vi "Color Steps Control.vi"(7 "Calling VI Ref":refnum<vi>) -> ()   [LabVIEW 2016]
uses:
  <vilib>/Utility/miscctls.llb/LVPointTypeDef.ctl
  Color Steps Type Def/Color Steps Presets Type.ctl
  Color Steps Type Def/Color Steps Step Type.ctl
  Laser Control/Laser Power Control/Laser Power Control Type Defs/Laser Power Ctrl Base Type.ctl
  Color Steps Type Def/Color Steps Notifier Type.ctl
  Color Steps Type Def/Color Step Actions.ctl
  Hardware Configuration/Hardware Configuration Controls/Device Type.ctl
  Hardware Configuration/Hardware Configuration Controls/Device Function.ctl
  Device Library/Filter Wheels/FW Type Defs/FW Actions.ctl
  Laser Control/Laser Power Control/Laser Power Control Type Defs/Laser Power Ctrl Messenger Actions.ctl
panel:
  in  "Tab Control":enum32{"Step Control", "Setup"}(tab)
  in  "Presets":u16(ring) items=["None"]
  in  "Step":T1(radio)
  in  "Add Step":bool
  in  "Update Step":bool
  in  "Remove Step":bool
  in  "Clear All":bool
  in  "Preset_Name":string
  in  "Step_Name_01":string
  in  "Step_Name_02":string
  in  "Step_Name_03":string
  in  "Step_Name_04":string
  in  "Step_Name_05":string
  in  "Save Preset":bool
  in  "Setup":bool=TRUE
  in  "Quit":bool
  # "Preset Name:"
  # "Step 01 Name:"
  # "Step 04 Name:"
  # "Step 02 Name:"
  # "Step 05 Name:"
  # "Step 03 Name:"
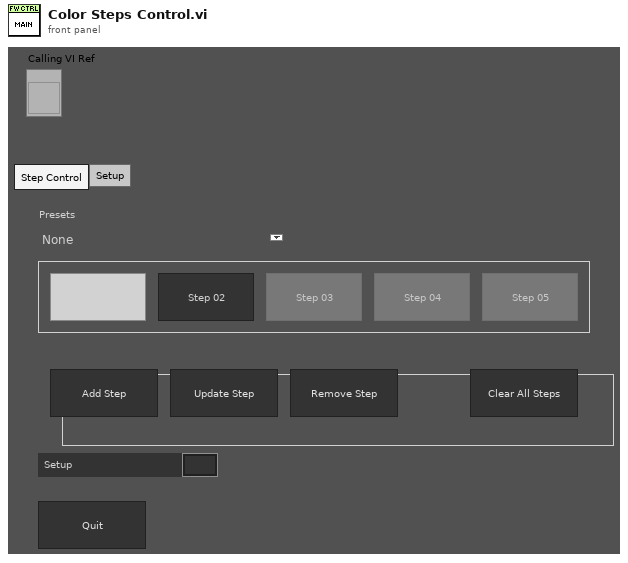
[diagram p1: front panel]
types:
  T1 = enum32{"Step 01", "Step 02", "Step 03", "Step 04", "Step 05"}
  T2 = typedef "Device Function.ctl" = enum16{"Primary", "Secondary", "Overview", "Wide Field Drift Correction", "642 nm Excitation", "560 nm Excitation", "940 nm Excitation", "546 nm Excitation", "488 nm Excitation", "405 nm Excitation", "Objective Drift Correction", "4Pi Objective Lock", "Objective XY", "Objective Z", "Sample XY", "Sample Coarse Z", "Sample Z", "4Pi Lower", "4Pi Upper", "Mojo", "Adj Cavity", "Line Scanning", "Alert"}
  T3 = typedef "Device Type.ctl" = enum16{"AOTF", "Camera", "Deformable Mirror", "Laser", "Shutter", "Stage", "Waveform", "FPGA", "Email", "Filter Wheel"}
  T4 = typedef "Color Steps Notifier Type.ctl" = cluster{"Actions":T5, "Set Step":i32, "Current Step":i32, "Last Step?":bool, "Received?":bool, "Preset Index":i32}
  T5 = typedef "Color Step Actions.ctl" = enum16{"Add Step", "Update Step", "Remove Step", "Clear All", "Get Status", "Next Step", "Go To Step", "Save Preset", "Change Preset", "Update Names", "Quit"}
  T6 = typedef "Color Steps Presets Type.ctl" = cluster{"Preset Name":string, "Steps":T7[]}
  T7 = typedef "Color Steps Step Type.ctl" = cluster{"Power Ctrl":T8[], "Filter Wheel Position":u8, "Step Name":string, "Wavelengths":u16[]}
  T8 = typedef "Laser Power Ctrl Base Type.ctl" = cluster{"Active":bool, "Power":dbl, "Ctrl Mode":u16}
  T9 = enum16{"Always On", "Always Off", "Off While Running"}
  T10 = typedef "LVPointTypeDef.ctl" = cluster{"Horizontal":i16, "Vertical":i16}
  T11 = enum8{"Enabled", "Disabled", "Disabled and Grayed Out"}
  T12 = typedef "LVRectTypeDef.ctl" = cluster{"Left":i16, "Top":i16, "Right":i16, "Bottom":i16}
  T13 = typedef "LVBoundsTypeDef.ctl" = cluster{"Width":u32, "Height":u32}
  T14 = typedef "Laser Power Ctrl Messenger Actions.ctl" = enum16{"All Active On", "All Off", "Adjust Power", "Line On/Off", "Get Status"}
  T15 = typedef "FW Actions.ctl" = enum16{"Set Position", "Get Position", "Get Num Positions", "Set Speed", "Quit"}
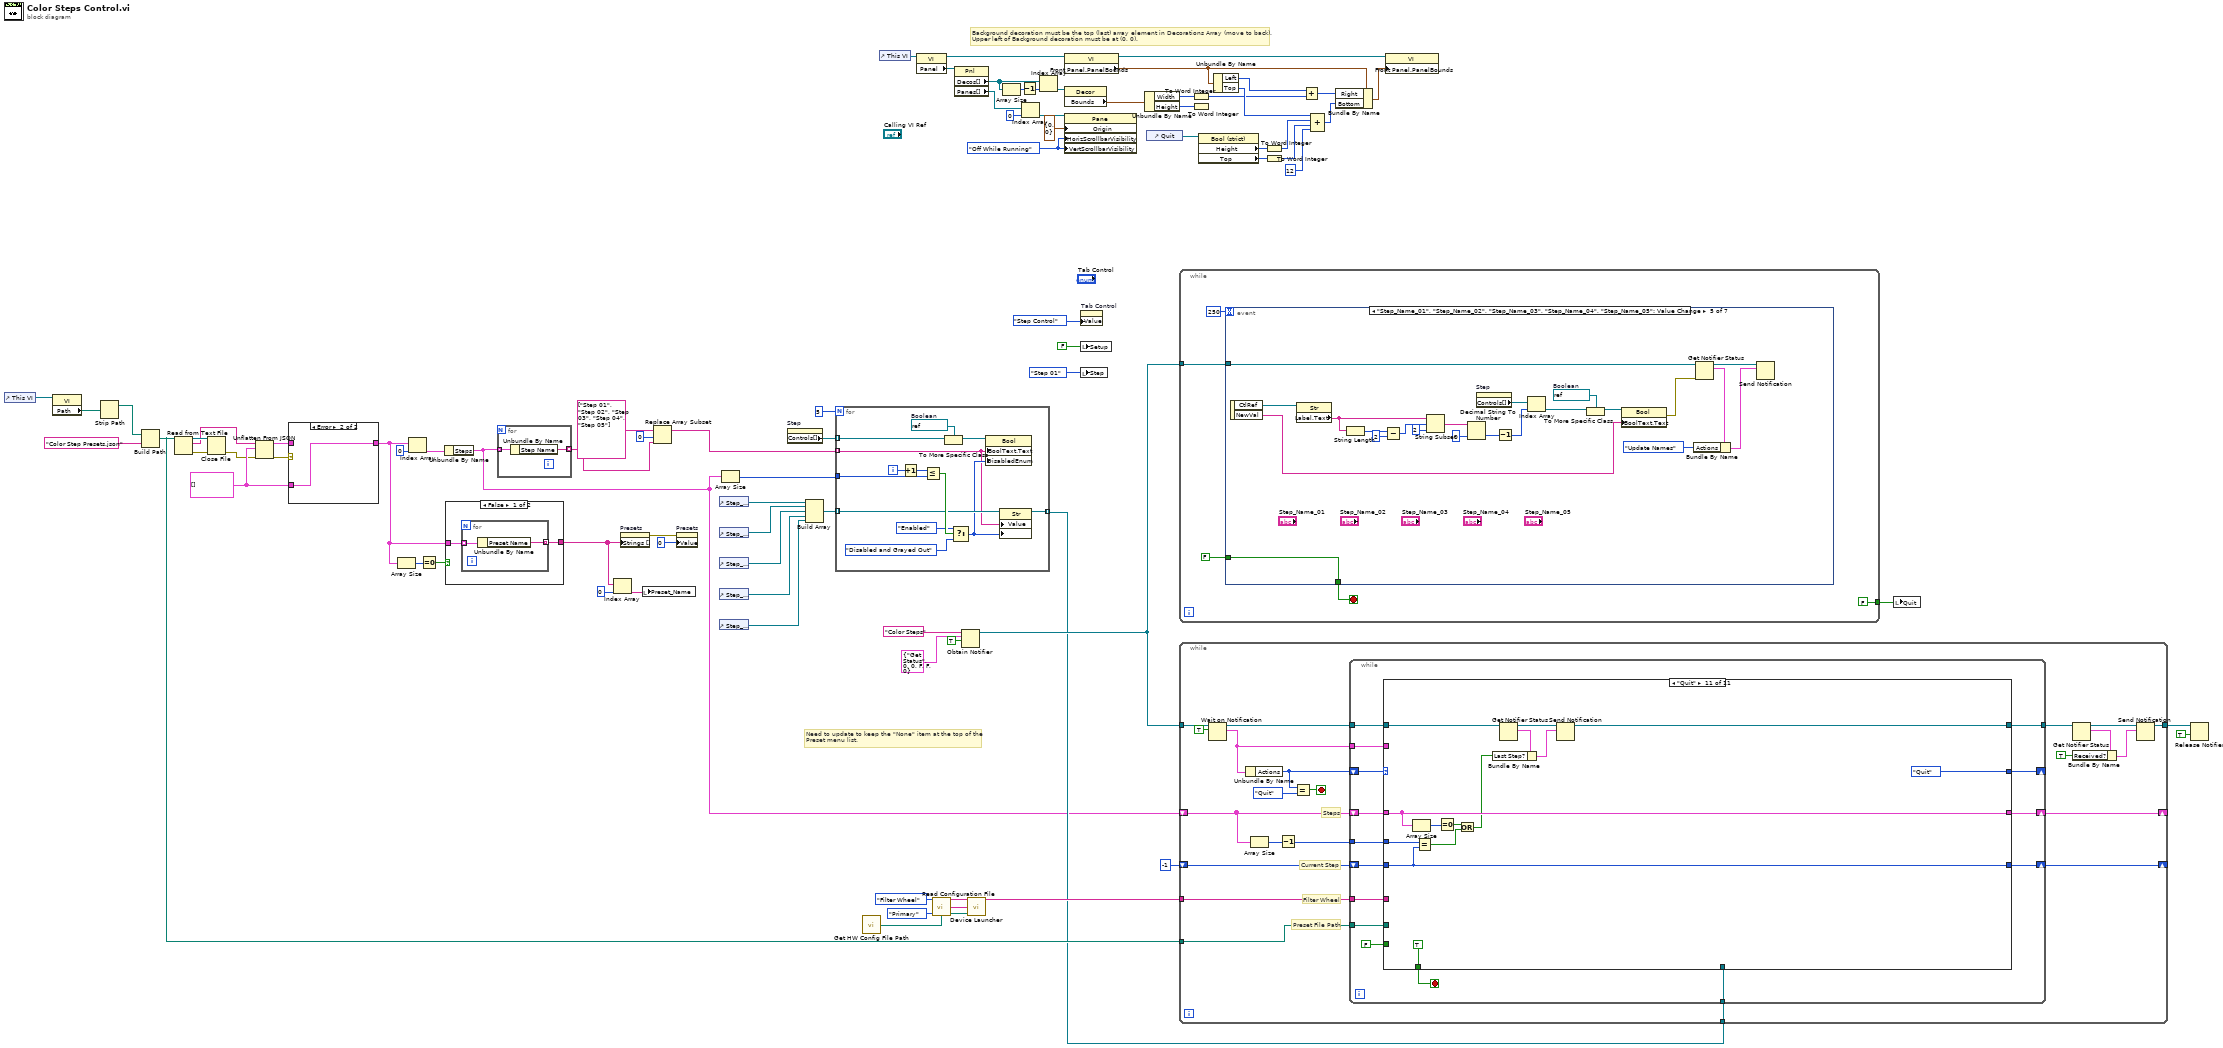
[diagram p0: block diagram]
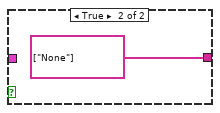
[diagram p2: hidden frame]
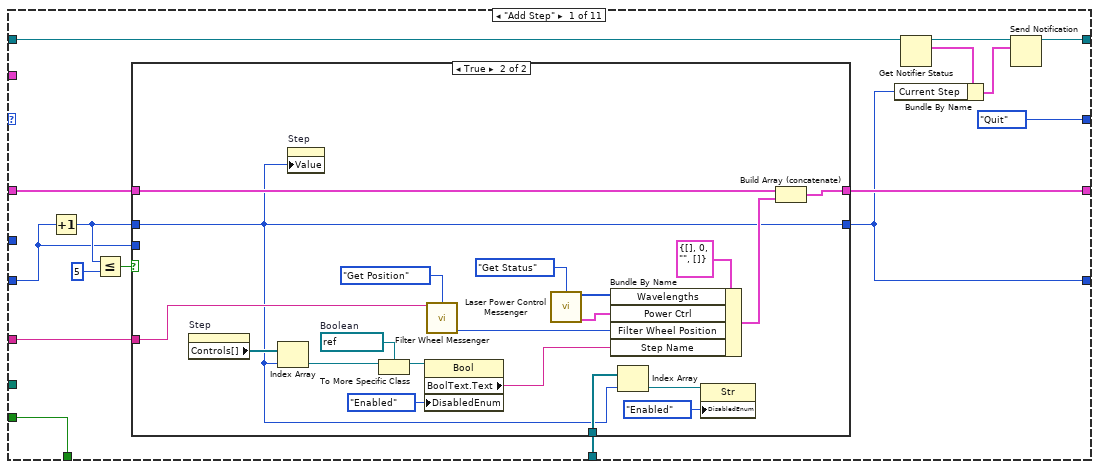
[diagram p3: hidden frame]
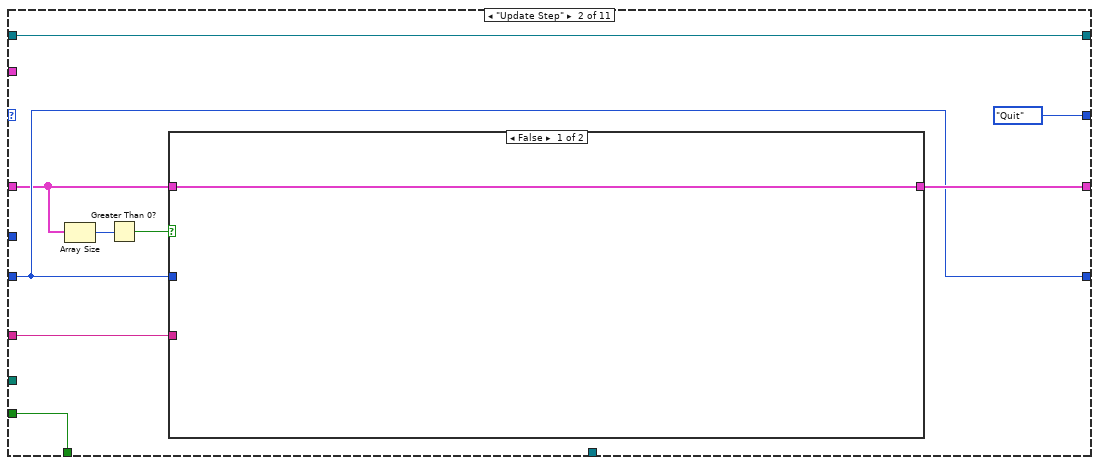
[diagram p5: hidden frame]
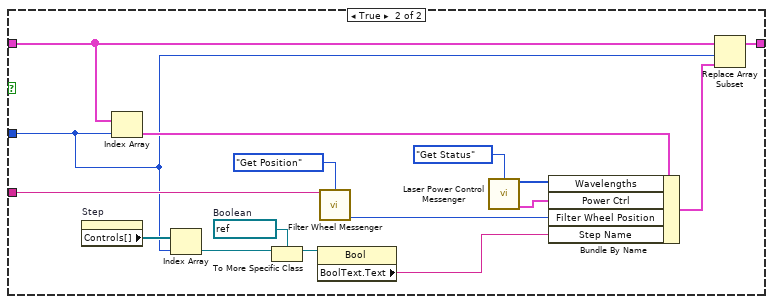
[diagram p6: hidden frame]
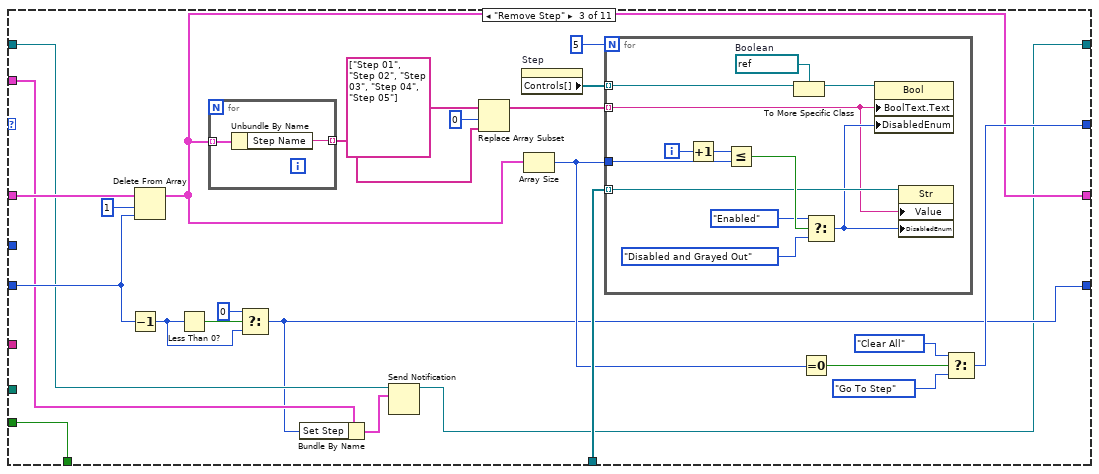
[diagram p7: hidden frame]
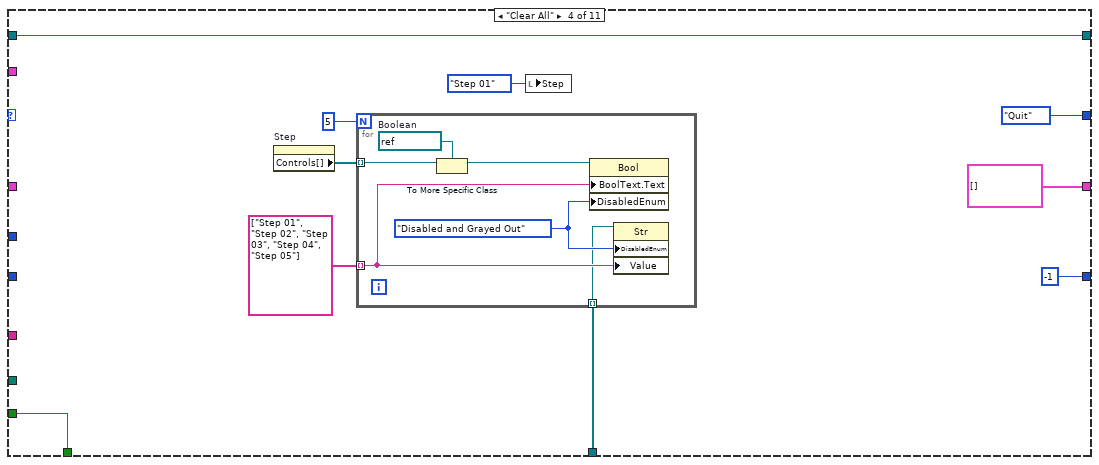
[diagram p8: hidden frame]
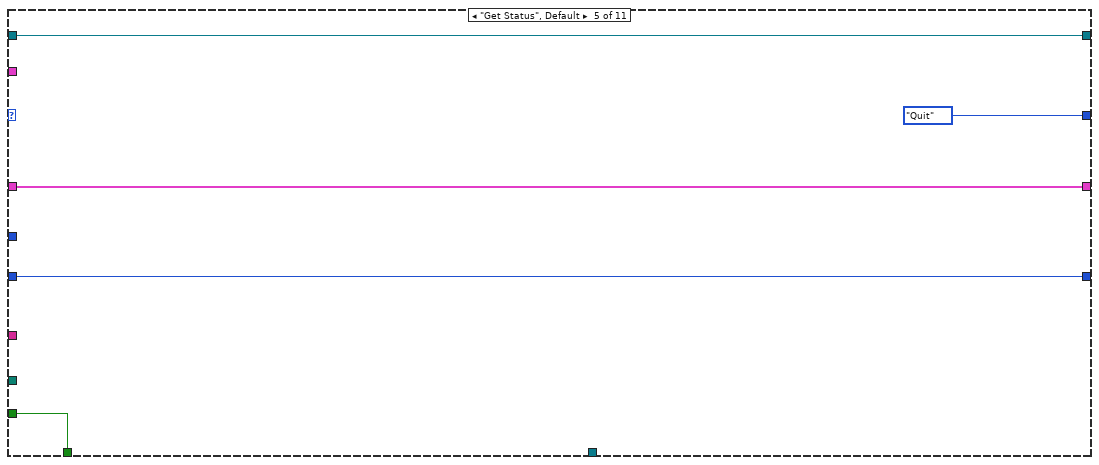
[diagram p9: hidden frame]
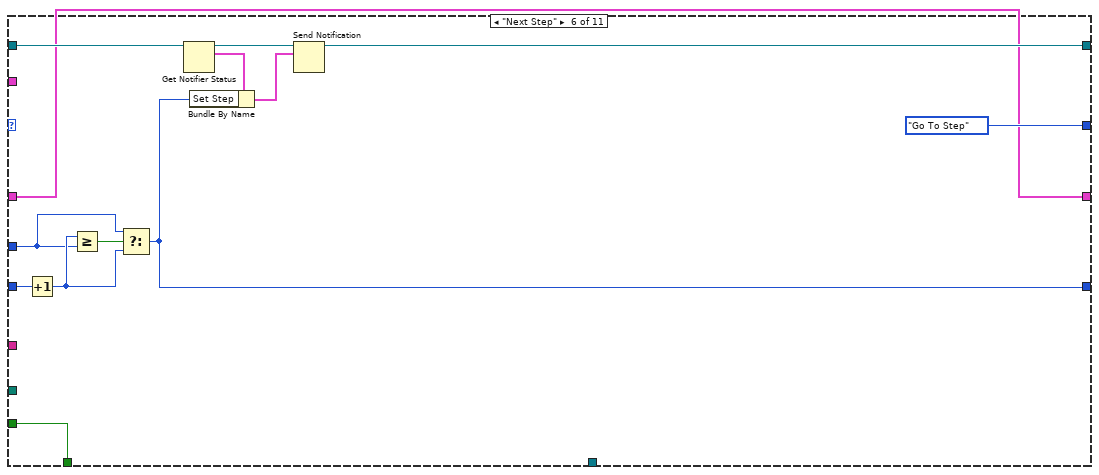
[diagram p10: hidden frame]
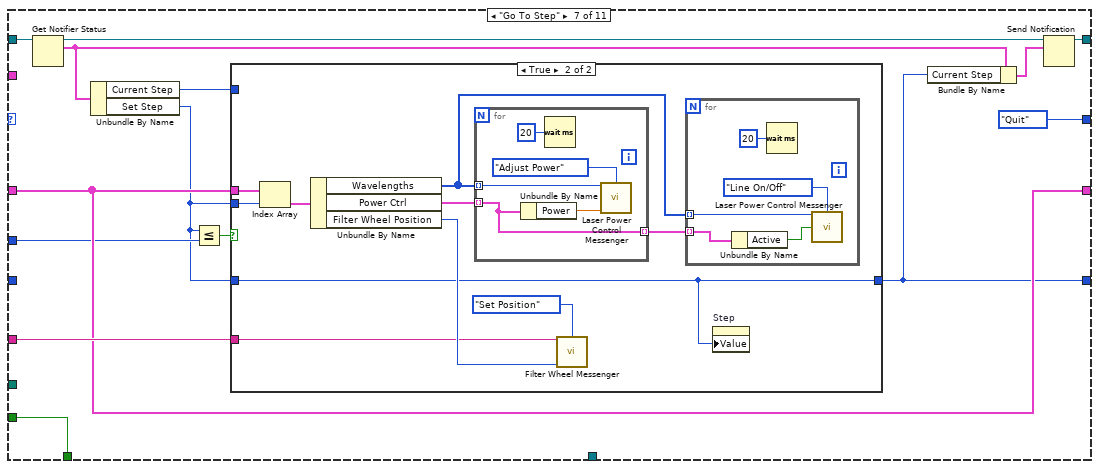
[diagram p11: hidden frame]
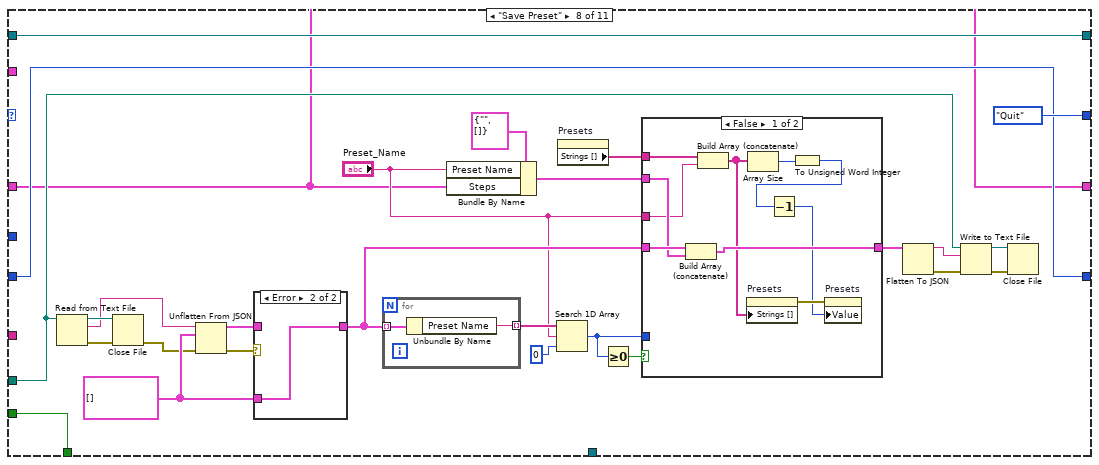
[diagram p13: hidden frame]
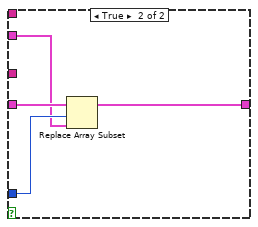
[diagram p14: hidden frame]
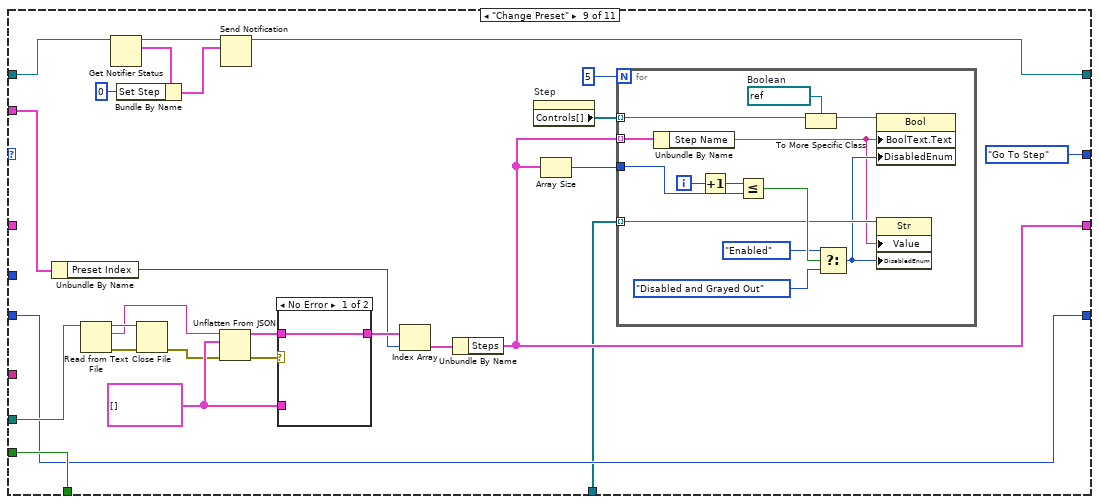
[diagram p16: hidden frame]
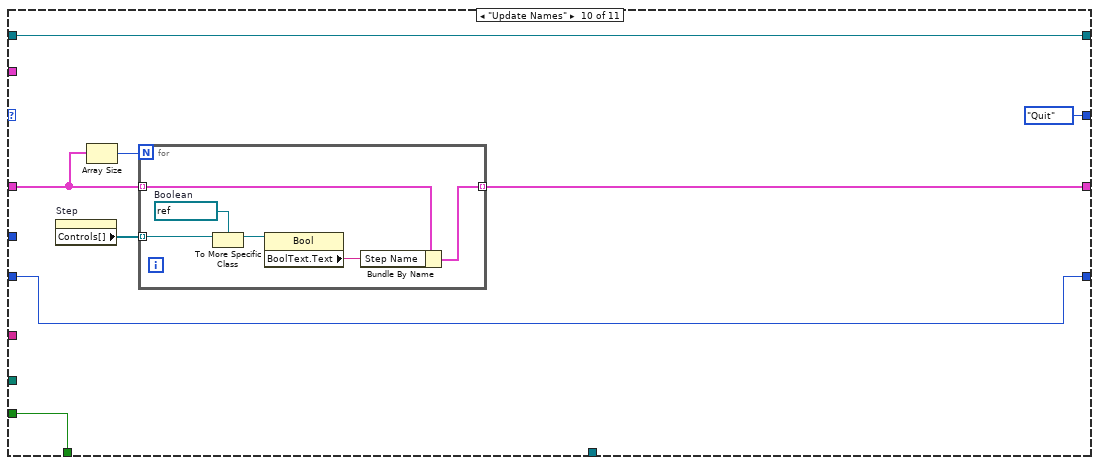
[diagram p18: hidden frame]
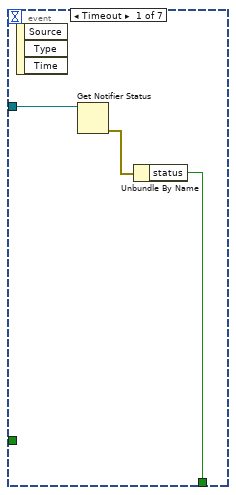
[diagram p19: hidden frame]
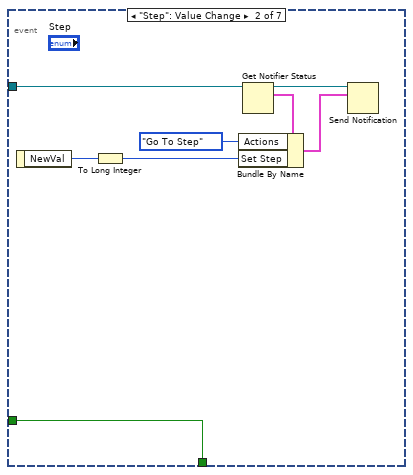
[diagram p20: hidden frame]
diagram:
  w40 = T6[] []
  w67 = T9."Off While Running" ("Vertical Scrollbar Visibility")
  # "Need to update to keep the \"None\" item at the top of the\nPreset menu list."
  # "Background decoration must be the top (last) array element in Decorations Array (move to back).\nUpper left of Background decoration must be at (0, 0)."
  n1 = control-ref of="This VI"() -> (w55:refnum<vi>)
  n2 = property class="VI"(reference=w55) -> ("Path"=w54:path)  [unwired: 1 in, 2 out]
  n3 = Strip Path(path=w54) -> (stripped path=w50:path)  [unwired: 1 out]
  n4 = Build Path(base path=w50, name or relative path="Color Step Presets.json") -> (appended path=w13:path)
  n5 = Read from Text File(file (use dialog)=w13) -> (refnum out=w39:refnum<file>, text=w36:string, error out=w38:errorcluster)  [unwired: 3 in, 1 out]
  n6 = Close File(refnum=w39, error in=w38) -> (error out=w37:errorcluster)  [unwired: 1 out]
  n7 = Unflatten From JSON(JSON string=w36, type and defaults=w40, error in (no error)=w37) -> (value=w51:T6[], error out=w52:errorcluster)  [unwired: 4 in]
  n8 = case shown="Error" w52 {
    tunnel: w51 -> [w85 _]
    tunnel: w40 -> [_ w86]
    tunnel: [w85 w86] -> w9
    frame No Error {
    }
    frame Error {
    }
  }
  n9 = Array Size(array=w9) -> (size(s)=w8:i32)
  n10 = Index Array(array=w9, index=0) -> (element=w23:T6)
  n11 = Equal To 0?(x=w8) -> (x = 0?=w7:bool)
  n12 = Unbundle By Name(w23) -> ("Steps"=w3:T7[])
  n13 = case shown="False" w7 {
    tunnel: w9 -> [w88 _]
    tunnel: [w87 string[] ["None"]] -> w11
    frame False {
      n14 = for {
        tunnel: w88 -> [w90] mode=indexing
        tunnel: [w89] -> w87 mode=indexing
        n15 = Unbundle By Name(w90) -> ("Preset Name"=w89:string)
      }
    }
    frame True {
    }
  }
  n16 = for {
    tunnel: w3 -> [w93] mode=indexing
    tunnel: [w92] -> w4 mode=indexing
    n17 = Unbundle By Name(w93) -> ("Step Name"=w92:string)
  }
  n18 = Index Array(array=w11, index=0) -> (element=w21:string)
  n19 = property on="Presets" class="Ring (strict)"("Strings []"=w11) -> (error out=w34:errorcluster)  [unwired: 2 in, 1 out]
  n20 = local write "Preset_Name"(w21) -> ()
  n21 = Replace Array Subset(array=string[] ["Step 01", "Step 02", "Step 03", "Step 04", "Step 05"], new element=w4, index=0) -> (w2:string[])
  n22 = property on="Presets" class="Ring (strict)"(error in=w34, "Value"=u16 0) -> ()  [unwired: 1 in, 2 out]
  n23 = control-ref of="Step_Name_01"() -> (w49:refnum<vi>)
  n24 = control-ref of="Step_Name_02"() -> (w45:refnum<vi>)
  n25 = control-ref of="Step_Name_03"() -> (w46:refnum<vi>)
  n26 = control-ref of="Step_Name_04"() -> (w47:refnum<vi>)
  n27 = control-ref of="Step_Name_05"() -> (w48:refnum<vi>)
  n28 = Array Size(array=w3) -> (size(s)=w32:i32)
  n29 = property on="Step" class="RadioBtnsControl (strict)"() -> ("Controls[]"=w43:refnum<vi>[])  [unwired: 2 in, 2 out]
  n30 = Build Array(w49, w45, w46, w47, w48) -> (w35:refnum<vi>[])
  n31 = for {
    N: 5 -> [_]
    tunnel: [w106] -> w12 mode=indexing
    tunnel: w43 -> [w105] mode=indexing
    tunnel: w35 -> [w97] mode=indexing
    tunnel: w32 -> [w96]
    tunnel: w2 -> [w94] mode=indexing
    i -> [w102]
    w104 = refnum<vi> refnum  # Boolean
    n32 = Increment(x=w102) -> (x+1=w101:i32)
    n33 = Less Or Equal?(x=w101, y=w96) -> (x <= y?=w100:bool)
    n34 = To More Specific Class(target class=w104, reference=w105) -> (specific class reference=w103:refnum<vi>)  [unwired: 1 in, 1 out]
    n35 = Select(t=T11."Enabled" ("Disabled"), s=w100, f=T11."Disabled and Grayed Out") -> (s? t:f=w95:T11)
    n36 = property class="Bool"(reference=w103, "BoolText.Text"=w94, "DisabledEnum"=w95) -> ()  [unwired: 1 in, 2 out]
    n37 = property class="Str"(reference=w97, "Value"=w94, "DisabledEnum"=w95) -> (reference out=w106:refnum<vi>)  [unwired: 1 in, 1 out]
  }
  n38 = call "Get HW Config File Path.vi"() -> ("File Path"=w15:path)  [unwired: 14 in, 1 out]
  n39 = control-ref of="This VI"() -> (w59:refnum<vi>)
  n40 = property class="VI"(reference=w59) -> (reference out=w68:refnum<vi>, "Panel"=w60:refnum<vi>)  [unwired: 1 in, 1 out]
  n41 = call "Read Configuration File.vi"("Device Type"=Device_Type."Filter Wheel", "Device Function"=Device_Function."Primary", "Config File Path"=w15) -> ("Unique Notifier Name"=w20:string, "Device Ports/IDs/Channels"=w18:string[], "Device Engine Path"=w19:path)  [unwired: 9 in, 1 out]
  n42 = property class="Pnl"(reference=w60) -> ("Decos[]"=w58:refnum<vi>[], "Panes[]"=w64:refnum<vi>[])  [unwired: 1 in, 2 out]
  n43 = Obtain Notifier(name (unnamed)="Color Steps", notification data type=T4 {"Actions"=enum."Get Status", "Set Step"=0, "Current Step"=0, "Last Step?"=FALSE, "Received?"=FALSE, "Preset Index"=0} ("Color Steps Note Type"), create if not found? (T)=TRUE) -> (notifier out=w27:refnum<notifier>)  [unwired: 1 in, 2 out]
  n44 = call "Device Launcher.vi"("Notifier Name"=w20, "Device Ports/IDs/Channels"=w18, "Device Engine Path"=w19) -> ("Notifier Name"=w14:string)  [unwired: 11 in, 1 out]
  n45 = Array Size(array=w58) -> (size(s)=w56:i32)
  n46 = Decrement(x=w56) -> (x-1=w57:i32)
  n47 = Index Array(array=w64, index=0) -> (element=w63:refnum<vi>)
  n48 = Index Array(array=w58, index=w57) -> (element=w66:refnum<vi>)
  n49 = property class="VI"(reference=w68) -> (reference out=w70:refnum<vi>, "Front Panel.PanelBounds"=w71:T12)  [unwired: 1 in, 1 out]
  n50 = property class="Decor"(reference=w66) -> ("Bounds"=w69:T13)  [unwired: 1 in, 2 out]
  n51 = property class="Pane"(reference=w63, "Origin"=T10 {"Horizontal"=0, "Vertical"=0}, "HorizScrollbarVisibility"=w67, "VertScrollbarVisibility"=w67) -> ()  [unwired: 1 in, 2 out]
  n52 = property on="Tab Control" class="TabCtl (strict)"("Value"=enum32{"Step Control", "Setup"}."Step Control" ("Tab Control")) -> ()  [unwired: 2 in, 2 out]
  n53 = local write "Setup"(FALSE ("Filter Wheel Setup")) -> ()
  n54 = local write "Step"(T1."Step 01" ("Step")) -> ()
  n55 = Unbundle By Name(w69) -> ("Width"=w74:u32, "Height"=w77:u32)
  n56 = control-ref of="Quit"() -> (w61:refnum<vi>)
  n57 = while {
    tunnel: w27 -> [w108]
    tunnel: [FALSE] -> w1
    stop <- w110 stop-if-true
    n58 = event shown="[4] \"Step_Name_01\", \"Step_Name_02\", \"Step_Name_03\", \"Step_Name_04\", \"Step_Name_05\": Value Change" {
      selector: _ -> [_ _ _ _ _ _ _]
      dyn-events: _ -> [_ _ _ _ _ _ _]
      timeout: 250 -> [_ _ _ _ _ _ _]
      tunnel: FALSE -> [_ w122 w130 w141 w163 w171 _]
      tunnel: [w112 w122 w130 w141 w163 w171 w177] -> w110
      tunnel: w108 -> [w114 w121 w124 _ w143 w166 w172]
      event Timeout {
        n59 = event-data() -> ()  [unwired: 1 in, 3 out]
        n60 = Get Notifier Status(notifier=w114) -> (error out=w113:errorcluster)  [unwired: 1 in, 4 out]
        n61 = Unbundle By Name(w113) -> ("status"=w112:bool)
      }
      event "Step": Value Change {
        n62 = event-data() -> ("NewVal"=w116:T1)  [unwired: 1 in]
        n63 = To Long Integer(number=w116) -> (32bit integer=w115:i32)
        n64 = Get Notifier Status(notifier=w121) -> (notifier out=w120:refnum<notifier>, current notification=w119:T4)  [unwired: 1 in, 3 out]
        n65 = Bundle By Name(cluster=w119, "Actions"=Color_Step_Actions."Go To Step", "Set Step"=w115) -> (w117:T4)
        n66 = Send Notification(notification=w117, notifier=w120) -> ()  [unwired: 1 in, 2 out]
      }
      event "Add Step", "Update Step", "Remove Step", "Clear All", "Save Preset": Value Change {
        n67 = event-data() -> ("CtlRef"=w129:refnum<vi>)  [unwired: 1 in]
        n68 = property class="Bool"(reference=w129) -> ("Label.Text"=w128:string)  [unwired: 1 in, 2 out]
        n69 = case shown="\"Add Step\"" w128 {
          tunnel: [Color_Step_Actions."Get Status" ("Actions") Color_Step_Actions."Add Step" ("Actions") Color_Step_Actions."Update Step" ("Actions") Color_Step_Actions."Remove Step" ("Actions") Color_Step_Actions."Clear All" ("Actions") Color_Step_Actions."Save Preset" ("Actions")] -> w123
          frame Default {
          }
          frame "Add Step" {
          }
          frame "Update Step" {
          }
          frame "Remove Step" {
          }
          frame "Clear All" {
          }
          frame "Save Preset" {
          }
        }
        n70 = Get Notifier Status(notifier=w124) -> (notifier out=w127:refnum<notifier>, current notification=w126:T4)  [unwired: 1 in, 3 out]
        n71 = Bundle By Name(cluster=w126, "Actions"=w123) -> (w125:T4)
        n72 = Send Notification(notification=w125, notifier=w127) -> ()  [unwired: 1 in, 2 out]
      }
      event "Setup": Value Change {
        n73 = event-data() -> ("NewVal"=w140:bool)  [unwired: 1 in]
        n74 = Select(t=enum32{"Step Control", "Setup"}."Setup" ("Tab Control"), s=w140, f=enum32{"Step Control", "Setup"}."Step Control" ("Tab Control")) -> (s? t:f=w137:enum32{"Step Control", "Setup"})
        n75 = property on="Tab Control" class="TabCtl (strict)"("Value"=w137) -> ()  [unwired: 2 in, 2 out]
      }
      event "Step_Name_01", "Step_Name_02", "Step_Name_03", "Step_Name_04", "Step_Name_05": Value Change {
        w162 = refnum<vi> refnum  # Boolean
        n76 = event-data() -> ("CtlRef"=w149:refnum<vi>, "NewVal"=w148:string)  [unwired: 1 in]
        n77 = property class="Str"(reference=w149) -> ("Label.Text"=w160:string)  [unwired: 1 in, 2 out]
        n78 = String Length(string=w160) -> (length=w159:i32)
        n79 = Subtract(x=w159, y=2) -> (x-y=w157:i32)
        n80 = String Subset(string=w160, offset (0)=w157, length (rest)=2 ("length (rest)")) -> (substring=w156:string)
        n81 = Decimal String To Number(string=w156, default (0L)=0 ("default (0 I32)")) -> (number=w153:i32)  [unwired: 1 in, 1 out]
        n82 = property on="Step" class="RadioBtnsControl (strict)"() -> ("Controls[]"=w154:refnum<vi>[])  [unwired: 2 in, 2 out]
        n83 = Decrement(x=w153) -> (x-1=w150:i32)
        n84 = Index Array(array=w154, index=w150) -> (element=w152:refnum<vi>)
        n85 = To More Specific Class(target class=w162, reference=w152) -> (specific class reference=w151:refnum<vi>)  [unwired: 1 in, 1 out]
        n86 = property class="Bool"(reference=w151, "BoolText.Text"=w148) -> (error out=w142:errorcluster)  [unwired: 1 in, 1 out]
        n87 = Get Notifier Status(notifier=w143, error in (no error)=w142) -> (notifier out=w147:refnum<notifier>, current notification=w146:T4)  [unwired: 3 out]
        n88 = Bundle By Name(cluster=w146, "Actions"=Color_Step_Actions."Update Names") -> (w144:T4)
        n89 = Send Notification(notification=w144, notifier=w147) -> ()  [unwired: 1 in, 2 out]
      }
      event "Presets": Value Change {
        n90 = event-data() -> ("NewVal"=w165:u16)  [unwired: 1 in]
        n91 = To Long Integer(number=w165) -> (32bit integer=w164:i32)
        n92 = Get Notifier Status(notifier=w166) -> (notifier out=w170:refnum<notifier>, current notification=w169:T4)  [unwired: 1 in, 3 out]
        n93 = Bundle By Name(cluster=w169, "Actions"=Color_Step_Actions."Change Preset", "Preset Index"=w164) -> (w167:T4)
        n94 = Send Notification(notification=w167, notifier=w170) -> ()  [unwired: 1 in, 2 out]
      }
      event "Quit": Value Change {
        n95 = event-data() -> ("NewVal"=w177:bool)  [unwired: 1 in]
        n96 = Get Notifier Status(notifier=w172) -> (notifier out=w176:refnum<notifier>, current notification=w175:T4)  [unwired: 1 in, 3 out]
        n97 = Bundle By Name(cluster=w175, "Actions"=Color_Step_Actions."Quit") -> (w173:T4)
        n98 = Send Notification(notification=w173, notifier=w176) -> ()  [unwired: 1 in, 2 out]
      }
    }
  }
  n99 = while {
    tunnel: w27 -> [w199]
    shift-right: [w185] -> _
    shift-left: w3 -> [w192]
    tunnel: [w178] -> w26
    shift-right: [w188] -> _
    shift-left: -1 -> [w193]
    tunnel: w14 -> [w189]
    tunnel: w13 -> [w187]
    tunnel: w12 -> [w184]
    stop <- w196 stop-if-true
    # "Preset File Path"
    # "Filter Wheel"
    # "Steps"
    # "Current Step"
    n100 = Wait on Notification(notifier=w199, ignore previous (F)=TRUE) -> (notifier out=w195:refnum<notifier>, notification=w186:T4)  [unwired: 2 in, 2 out]
    n101 = Unbundle By Name(w186) -> ("Actions"=w194:T5)
    n102 = Array Size(array=w192) -> (size(s)=w191:i32)
    n103 = Decrement(x=w191) -> (x-1=w190:i32)
    n104 = Equal?(x=w194, y=Color_Step_Actions."Quit") -> (x = y?=w196:bool)
    n105 = while {
      tunnel: w195 -> [w214]
      shift-right: [w206] -> _
      shift-left: w194 -> [w213]
      shift-right: [w201] -> w188
      shift-left: w193 -> [w208]
      shift-right: [w203] -> w185
      shift-left: w192 -> [w209]
      tunnel: w190 -> [w210]
      tunnel: w189 -> [w207]
      tunnel: w187 -> [w205]
      tunnel: w186 -> [w204]
      tunnel: w184 -> [w202]
      tunnel: [w200] -> w179
      stop <- w211 stop-if-true
      n106 = case shown="\"Quit\"" w213 {
        tunnel: w214 -> [w222 w256 w282 w326 w337 w346 w354 w390 w434 w479 w495]
        tunnel: FALSE -> [w230 w261 w303 w327 w338 w351 w365 w413 w457 w480 _]
        tunnel: [w230 w261 w303 w327 w338 w351 w365 w413 w457 w480 TRUE] -> w211
        tunnel: [w221 w256 w279 w326 w337 w345 w362 w390 w432 w479 w494] -> w200
        tunnel: w210 -> [_ _ _ _ _ w341 w359 _ _ _ w493]
        tunnel: w209 -> [w229 w255 w302 _ w334 w340 w360 w387 _ w476 w491]
        tunnel: w208 -> [w216 w258 w300 _ w336 w350 _ w392 w444 w473 w492]
        tunnel: w207 -> [w226 w260 _ _ _ _ w364 _ _ _ _]
        tunnel: [w220 w258 w280 -1 ("Set Step") w336 w339 w355 w392 w444 w473 w492] -> w201
        tunnel: [Color_Step_Actions."Quit" ("y") Color_Step_Actions."Quit" ("y") w287 Color_Step_Actions."Quit" ("y") Color_Step_Actions."Quit" ("y") Color_Step_Actions."Go To Step" ("y") Color_Step_Actions."Quit" ("y") Color_Step_Actions."Quit" ("y") Color_Step_Actions."Go To Step" ("y") Color_Step_Actions."Quit" ("y") Color_Step_Actions."Quit" ("y")] -> w206
        tunnel: w205 -> [_ _ _ _ _ _ _ w395 w449 _ _]
        tunnel: w204 -> [_ _ w283 _ _ _ _ _ w448 _ _]
        tunnel: [w227 w259 w286 T7[] [] ("Steps") w334 w340 w360 w387 w440 w477 w491] -> w203
        tunnel: w202 -> [w215 _ w295 w320 _ _ _ _ w438 _ _]
        frame "Add Step" {
          n107 = Increment(x=w216) -> (x+1=w218:i32)
          n108 = Less Or Equal?(x=w218, y=5) -> (x <= y?=w219:bool)
          n109 = case shown="True" w219 {
            tunnel: w229 -> [w232 w252]
            tunnel: [w232 w251] -> w227
            tunnel: w226 -> [_ w240]
            tunnel: w218 -> [_ w233]
            tunnel: [w231 w233] -> w220
            tunnel: w216 -> [w231 _]
            tunnel: w215 -> [_ w236]
            frame False {
            }
            frame True {
              w249 = refnum<vi> refnum  # Boolean
              n110 = property on="Step" class="RadioBtnsControl (strict)"() -> ("Controls[]"=w250:refnum<vi>[])  [unwired: 2 in, 2 out]
              n111 = Index Array(array=w250, index=w233) -> (element=w248:refnum<vi>)
              n112 = property on="Step" class="RadioBtnsControl (strict)"("Value"=w233) -> ()  [unwired: 2 in, 2 out]
              n113 = To More Specific Class(target class=w249, reference=w248) -> (specific class reference=w247:refnum<vi>)  [unwired: 1 in, 1 out]
              n114 = property class="Bool"(reference=w247, "DisabledEnum"=T11."Enabled" ("Disabled")) -> ("BoolText.Text"=w246:string)  [unwired: 1 in, 2 out]
              n115 = call "Filter Wheel Messenger.vi"("FW Notifier"=w240, "Actions"=FW_Actions."Get Position") -> ("Current Position"=w244:u8)  [unwired: 11 in, 2 out]
              n116 = call "Laser Power Control Messenger.vi"("Power Ctrl Actions"=Laser_Power_Ctrl_Messenger_Actions."Get Status") -> ("Wavelengths"=w242:u16[], "Power Status"=w241:T8[])  [unwired: 13 in]
              n117 = Bundle By Name(cluster=T7 {"Power Ctrl"=[], "Filter Wheel Position"=0, "Step Name"="", "Wavelengths"=[]} ("Step"), "Wavelengths"=w242, "Power Ctrl"=w241, "Filter Wheel Position"=w244, "Step Name"=w246) -> (w238:T7)
              n118 = Index Array(array=w236, index=w233) -> (element=w235:refnum<vi>)
              n119 = property class="Str"(reference=w235, "DisabledEnum"=T11."Enabled" ("Disabled")) -> ()  [unwired: 1 in, 2 out]
              n120 = Build Array (concatenate)(w252, w238) -> (w251:T7[])
            }
          }
          n121 = Get Notifier Status(notifier=w222) -> (notifier out=w223:refnum<notifier>, current notification=w224:T4)  [unwired: 1 in, 3 out]
          n122 = Bundle By Name(cluster=w224, "Current Step"=w220) -> (w225:T4)
          n123 = Send Notification(notification=w225, notifier=w223) -> (notifier out=w221:refnum<notifier>)  [unwired: 1 in, 1 out]
        }
        frame "Update Step" {
          n124 = Array Size(array=w255) -> (size(s)=w254:i32)
          n125 = Greater Than 0?(x=w254) -> (x > 0?=w253:bool)
          n126 = case shown="False" w253 {
            tunnel: w260 -> [_ w270]
            tunnel: [w262 w265] -> w259
            tunnel: w258 -> [_ w264]
            tunnel: w255 -> [w262 w263]
            frame False {
            }
            frame True {
              w275 = refnum<vi> refnum  # Boolean
              n127 = property on="Step" class="RadioBtnsControl (strict)"() -> ("Controls[]"=w276:refnum<vi>[])  [unwired: 2 in, 2 out]
              n128 = Index Array(array=w263, index=w264) -> (element=w278:T7)
              n129 = Index Array(array=w276, index=w264) -> (element=w274:refnum<vi>)
              n130 = To More Specific Class(target class=w275, reference=w274) -> (specific class reference=w273:refnum<vi>)  [unwired: 1 in, 1 out]
              n131 = property class="Bool"(reference=w273) -> ("BoolText.Text"=w272:string)  [unwired: 1 in, 2 out]
              n132 = call "Filter Wheel Messenger.vi"("FW Notifier"=w270, "Actions"=FW_Actions."Get Position") -> ("Current Position"=w269:u8)  [unwired: 11 in, 2 out]
              n133 = call "Laser Power Control Messenger.vi"("Power Ctrl Actions"=Laser_Power_Ctrl_Messenger_Actions."Get Status") -> ("Wavelengths"=w267:u16[], "Power Status"=w266:T8[])  [unwired: 13 in]
              n134 = Bundle By Name(cluster=w278, "Wavelengths"=w267, "Power Ctrl"=w266, "Filter Wheel Position"=w269, "Step Name"=w272) -> (w277:T7)
              n135 = Replace Array Subset(array=w263, new element=w277, index=w264) -> (w265:T7[])
            }
          }
        }
        frame "Remove Step" {
          n136 = Decrement(x=w300) -> (x-1=w299:i32)
          n137 = Delete From Array(array=w302, length=1, index=w300) -> (array with subset deleted=w286:T7[])  [unwired: 1 out]
          n138 = Less Than 0?(x=w299) -> (x < 0?=w288:bool)
          n139 = for {
            tunnel: w286 -> [w305] mode=indexing
            tunnel: [w304] -> w292 mode=indexing
            n140 = Unbundle By Name(w305) -> ("Step Name"=w304:string)
          }
          n141 = Select(t=0, s=w288, f=w299) -> (s? t:f=w280:i32)
          n142 = Bundle By Name(cluster=w283, "Set Step"=w280) -> (w281:T4)
          n143 = Send Notification(notification=w281, notifier=w282) -> (notifier out=w279:refnum<notifier>)  [unwired: 1 in, 1 out]
          n144 = Replace Array Subset(array=string[] ["Step 01", "Step 02", "Step 03", "Step 04", "Step 05"], new element=w292, index=0) -> (w291:string[])
          n145 = property on="Step" class="RadioBtnsControl (strict)"() -> ("Controls[]"=w296:refnum<vi>[])  [unwired: 2 in, 2 out]
          n146 = Array Size(array=w286) -> (size(s)=w285:i32)
          n147 = for {
            N: 5 -> [_]
            tunnel: w296 -> [w317] mode=indexing
            tunnel: w295 -> [w309] mode=indexing
            tunnel: w285 -> [w308]
            tunnel: w291 -> [w306] mode=indexing
            i -> [w314]
            w316 = refnum<vi> refnum  # Boolean
            n148 = Increment(x=w314) -> (x+1=w313:i32)
            n149 = Less Or Equal?(x=w313, y=w308) -> (x <= y?=w312:bool)
            n150 = To More Specific Class(target class=w316, reference=w317) -> (specific class reference=w315:refnum<vi>)  [unwired: 1 in, 1 out]
            n151 = Select(t=T11."Enabled" ("Disabled"), s=w312, f=T11."Disabled and Grayed Out") -> (s? t:f=w307:T11)
            n152 = property class="Bool"(reference=w315, "BoolText.Text"=w306, "DisabledEnum"=w307) -> ()  [unwired: 1 in, 2 out]
            n153 = property class="Str"(reference=w309, "Value"=w306, "DisabledEnum"=w307) -> ()  [unwired: 1 in, 2 out]
          }
          n154 = Equal To 0?(x=w285) -> (x = 0?=w284:bool)
          n155 = Select(t=Color_Step_Actions."Clear All" ("y"), s=w284, f=Color_Step_Actions."Go To Step" ("y")) -> (s? t:f=w287:T5)
        }
        frame "Clear All" {
          n156 = property on="Step" class="RadioBtnsControl (strict)"() -> ("Controls[]"=w322:refnum<vi>[])  [unwired: 2 in, 2 out]
          n157 = for {
            N: 5 -> [_]
            tunnel: w322 -> [w333] mode=indexing
            tunnel: string[] ["Step 01", "Step 02", "Step 03", "Step 04", "Step 05"] -> [w329] mode=indexing
            tunnel: w320 -> [w328] mode=indexing
            w330 = T11."Disabled and Grayed Out" ("f")
            w332 = refnum<vi> refnum  # Boolean
            n158 = To More Specific Class(target class=w332, reference=w333) -> (specific class reference=w331:refnum<vi>)  [unwired: 1 in, 1 out]
            n159 = property class="Bool"(reference=w331, "BoolText.Text"=w329, "DisabledEnum"=w330) -> ()  [unwired: 1 in, 2 out]
            n160 = property class="Str"(reference=w328, "DisabledEnum"=w330, "Value"=w329) -> ()  [unwired: 1 in, 2 out]
          }
          n161 = local write "Step"(T1."Step 01" ("Step")) -> ()
        }
        frame "Get Status", Default {
        }
        frame "Next Step" {
          n162 = Increment(x=w350) -> (x+1=w343:i32)
          n163 = Greater Or Equal?(x=w343, y=w341) -> (x >= y?=w342:bool)
          n164 = Select(t=w341, s=w342, f=w343) -> (s? t:f=w339:i32)
          n165 = Get Notifier Status(notifier=w346) -> (notifier out=w347:refnum<notifier>, current notification=w348:T4)  [unwired: 1 in, 3 out]
          n166 = Bundle By Name(cluster=w348, "Set Step"=w339) -> (w349:T4)
          n167 = Send Notification(notification=w349, notifier=w347) -> (notifier out=w345:refnum<notifier>)  [unwired: 1 in, 1 out]
        }
        frame "Go To Step" {
          n168 = Get Notifier Status(notifier=w354) -> (notifier out=w353:refnum<notifier>, current notification=w352:T4)  [unwired: 1 in, 3 out]
          n169 = Unbundle By Name(w352) -> ("Current Step"=w356:i32, "Set Step"=w357:i32)
          n170 = Less Or Equal?(x=w357, y=w359) -> (x <= y?=w358:bool)
          n171 = case shown="True" w358 {
            tunnel: w364 -> [_ w370]
            tunnel: w357 -> [_ w369]
            tunnel: w360 -> [_ w368]
            tunnel: w357 -> [_ w367]
            tunnel: [w366 w367] -> w355
            tunnel: w356 -> [w366 _]
            frame False {
            }
            frame True {
              n172 = Index Array(array=w368, index=w369) -> (element=w371:T7)
              n173 = Unbundle By Name(w371) -> ("Wavelengths"=w376:u16[], "Power Ctrl"=w374:T8[], "Filter Wheel Position"=w373:u8)
              n174 = for {
                tunnel: w374 -> [w383] mode=indexing
                tunnel: w376 -> [w384] mode=indexing
                tunnel: [w383] -> w375 mode=indexing
                n175 = Unbundle By Name(w383) -> ("Power"=w385:dbl)
                n176 = Wait (ms)(milliseconds to wait=u32 20) -> ()  [unwired: 1 out]
                n177 = call "Laser Power Control Messenger.vi"("Wavelength (nm)"=w384, "Power Ctrl Actions"=Laser_Power_Ctrl_Messenger_Actions."Adjust Power", "Power"=w385) -> ()  [unwired: 11 in, 2 out]
              }
              n178 = call "Filter Wheel Messenger.vi"("FW Notifier"=w370, "Actions"=FW_Actions."Set Position", "Set Position"=w373) -> ()  [unwired: 10 in, 3 out]
              n179 = for {
                tunnel: w375 -> [w379] mode=indexing
                tunnel: w376 -> [w380] mode=indexing
                n180 = Unbundle By Name(w379) -> ("Active"=w378:bool)
                n181 = Wait (ms)(milliseconds to wait=u32 20) -> ()  [unwired: 1 out]
                n182 = call "Laser Power Control Messenger.vi"("Wavelength (nm)"=w380, "Power Ctrl Actions"=Laser_Power_Ctrl_Messenger_Actions."Line On/Off", "Line On/Off"=w378) -> ()  [unwired: 11 in, 2 out]
              }
              n183 = property on="Step" class="RadioBtnsControl (strict)"("Value"=w367) -> ()  [unwired: 2 in, 2 out]
            }
          }
          n184 = Bundle By Name(cluster=w352, "Current Step"=w355) -> (w363:T4)
          n185 = Send Notification(notification=w363, notifier=w353) -> (notifier out=w362:refnum<notifier>)  [unwired: 1 in, 1 out]
        }
        frame "Save Preset" {
          w409 = T6[] []
          n186 = Read from Text File(file (use dialog)=w395) -> (refnum out=w408:refnum<file>, text=w405:string, error out=w407:errorcluster)  [unwired: 3 in, 1 out]
          n187 = Close File(refnum=w408, error in=w407) -> (error out=w406:errorcluster)  [unwired: 1 out]
          n188 = Unflatten From JSON(JSON string=w405, type and defaults=w409, error in (no error)=w406) -> (value=w410:T6[], error out=w411:errorcluster)  [unwired: 4 in]
          n189 = case shown="Error" w411 {
            tunnel: w410 -> [w430 _]
            tunnel: w409 -> [_ w431]
            tunnel: [w430 w431] -> w401
            frame No Error {
            }
            frame Error {
            }
          }
          n190 = for {
            tunnel: w401 -> [w429] mode=indexing
            tunnel: [w428] -> w404 mode=indexing
            n191 = Unbundle By Name(w429) -> ("Preset Name"=w428:string)
          }
          n192 = Bundle By Name(cluster=T6 {"Preset Name"="", "Steps"=[]} ("Presets"), "Preset Name"="Preset_Name", "Steps"=w387) -> (w399:T6)
          n193 = Search 1D Array(1D array=w404, element="Preset_Name", start index (0)=0) -> (index of element=w402:i32)
          n194 = property on="Presets" class="Ring (strict)"() -> ("Strings []"=w389:string[])  [unwired: 2 in, 2 out]
          n195 = Greater Or Equal To 0?(x=w402) -> (x >= 0?=w403:bool)
          n196 = case shown="False" w403 {
            tunnel: w402 -> [_ w426]
            tunnel: w401 -> [w423 w427]
            tunnel: w399 -> [w422 w424]
            tunnel: [w421 w425] -> w398
            tunnel: w389 -> [w420 _]
            tunnel: "Preset_Name" -> [w419 _]
            frame False {
              n197 = Build Array (concatenate)(w423, w422) -> (w421:T6[])
              n198 = Build Array (concatenate)(w420, w419) -> (w417:string[])
              n199 = property on="Presets" class="Ring (strict)"("Strings []"=w417) -> (error out=w418:errorcluster)  [unwired: 2 in, 1 out]
              n200 = Array Size(array=w417) -> (size(s)=w416:i32)
              n201 = To Unsigned Word Integer(number=w416) -> (unsigned 16bit integer=w415:u16)
              n202 = Decrement(x=w415) -> (x-1=w414:u16)
              n203 = property on="Presets" class="Ring (strict)"(error in=w418, "Value"=w414) -> ()  [unwired: 1 in, 2 out]
            }
            frame True {
              n204 = Replace Array Subset(array=w427, new element=w424, index=w426) -> (w425:T6[])
            }
          }
          n205 = Flatten To JSON(anything=w398) -> (JSON string=w397:string, 11:w396:errorcluster)  [unwired: 2 in]
          n206 = Write to Text File(file (use dialog)=w395, text=w397, error in=w396) -> (refnum out=w394:refnum<file>, error out=w393:errorcluster)  [unwired: 1 in, 1 out]
          n207 = Close File(refnum=w394, error in=w393) -> ()  [unwired: 2 out]
        }
        frame "Change Preset" {
          w454 = T6[] []
          n208 = Unbundle By Name(w448) -> ("Preset Index"=w446:i32)
          n209 = Read from Text File(file (use dialog)=w449) -> (refnum out=w453:refnum<file>, text=w450:string, error out=w452:errorcluster)  [unwired: 3 in, 1 out]
          n210 = Get Notifier Status(notifier=w434) -> (notifier out=w435:refnum<notifier>, current notification=w436:T4)  [unwired: 1 in, 3 out]
          n211 = Bundle By Name(cluster=w436, "Set Step"=0) -> (w437:T4)
          n212 = Close File(refnum=w453, error in=w452) -> (error out=w451:errorcluster)  [unwired: 1 out]
          n213 = Unflatten From JSON(JSON string=w450, type and defaults=w454, error in (no error)=w451) -> (value=w455:T6[], error out=w456:errorcluster)  [unwired: 4 in]
          n214 = Send Notification(notification=w437, notifier=w435) -> (notifier out=w432:refnum<notifier>)  [unwired: 1 in, 1 out]
          n215 = case shown="No Error" w456 {
            tunnel: w455 -> [w471 _]
            tunnel: w454 -> [_ w472]
            tunnel: [w471 w472] -> w447
            frame No Error {
            }
            frame Error {
            }
          }
          n216 = Index Array(array=w447, index=w446) -> (element=w445:T6)
          n217 = Unbundle By Name(w445) -> ("Steps"=w440:T7[])
          n218 = property on="Step" class="RadioBtnsControl (strict)"() -> ("Controls[]"=w442:refnum<vi>[])  [unwired: 2 in, 2 out]
          n219 = Array Size(array=w440) -> (size(s)=w439:i32)
          n220 = for {
            N: 5 -> [_]
            tunnel: w442 -> [w470] mode=indexing
            tunnel: w438 -> [w462] mode=indexing
            tunnel: w439 -> [w461]
            tunnel: w440 -> [w459] mode=indexing
            i -> [w467]
            w469 = refnum<vi> refnum  # Boolean
            n221 = Unbundle By Name(w459) -> ("Step Name"=w458:string)
            n222 = Increment(x=w467) -> (x+1=w466:i32)
            n223 = Less Or Equal?(x=w466, y=w461) -> (x <= y?=w465:bool)
            n224 = To More Specific Class(target class=w469, reference=w470) -> (specific class reference=w468:refnum<vi>)  [unwired: 1 in, 1 out]
            n225 = Select(t=T11."Enabled" ("Disabled"), s=w465, f=T11."Disabled and Grayed Out") -> (s? t:f=w460:T11)
            n226 = property class="Bool"(reference=w468, "BoolText.Text"=w458, "DisabledEnum"=w460) -> ()  [unwired: 1 in, 2 out]
            n227 = property class="Str"(reference=w462, "Value"=w458, "DisabledEnum"=w460) -> ()  [unwired: 1 in, 2 out]
          }
        }
        frame "Update Names" {
          n228 = property on="Step" class="RadioBtnsControl (strict)"() -> ("Controls[]"=w474:refnum<vi>[])  [unwired: 2 in, 2 out]
          n229 = Array Size(array=w476) -> (size(s)=w475:i32)
          n230 = for {
            N: w475 -> [_]
            tunnel: w476 -> [w486] mode=indexing
            tunnel: [w482] -> w477 mode=indexing
            tunnel: w474 -> [w481] mode=indexing
            w484 = refnum<vi> refnum  # Boolean
            n231 = To More Specific Class(target class=w484, reference=w481) -> (specific class reference=w485:refnum<vi>)  [unwired: 1 in, 1 out]
            n232 = property class="Bool"(reference=w485) -> ("BoolText.Text"=w483:string)  [unwired: 1 in, 2 out]
            n233 = Bundle By Name(cluster=w486, "Step Name"=w483) -> (w482:T7)
          }
        }
        frame "Quit" {
          n234 = Array Size(array=w491) -> (size(s)=w490:i32)
          n235 = Equal?(x=w493, y=w492) -> (x = y?=w488:bool)
          n236 = Equal To 0?(x=w490) -> (x = 0?=w489:bool)
          n237 = Or(x=w489, y=w488) -> (x .or. y?=w487:bool)
          n238 = Get Notifier Status(notifier=w495) -> (notifier out=w496:refnum<notifier>, current notification=w497:T4)  [unwired: 1 in, 3 out]
          n239 = Bundle By Name(cluster=w497, "Last Step?"=w487) -> (w498:T4)
          n240 = Send Notification(notification=w498, notifier=w496) -> (notifier out=w494:refnum<notifier>)  [unwired: 1 in, 1 out]
        }
      }
    }
    n241 = Get Notifier Status(notifier=w179) -> (notifier out=w183:refnum<notifier>, current notification=w182:T4)  [unwired: 1 in, 3 out]
    n242 = Bundle By Name(cluster=w182, "Received?"=TRUE) -> (w180:T4)
    n243 = Send Notification(notification=w180, notifier=w183) -> (notifier out=w178:refnum<notifier>)  [unwired: 1 in, 1 out]
  }
  n244 = To Word Integer(number=w74) -> (16bit integer=w76:i16)
  n245 = To Word Integer(number=w77) -> ()  [unwired: 1 out]
  n246 = property class="Bool (strict)"(reference=w61) -> ("Height"=w79:u32, "Top"=w80:i32)  [unwired: 1 in, 2 out]
  n247 = Unbundle By Name(w71) -> ("Left"=w73:i16, "Top"=w84:i16)
  n248 = To Word Integer(number=w79) -> (16bit integer=w82:i16)
  n249 = To Word Integer(number=w80) -> (16bit integer=w83:i16)
  n250 = Add(x=w73, y=w76) -> (x+y=w75:i16)
  n251 = Compound Arithmetic op=ADD(w84, w82, w83, i16 12 ("y")) -> (w78:i16)
  n252 = Bundle By Name(cluster=w71, "Right"=w75, "Bottom"=w78) -> (w72:T12)
  n253 = property class="VI"(reference=w70, "Front Panel.PanelBounds"=w72) -> ()  [unwired: 1 in, 2 out]
  n254 = local write "Quit"(w1) -> ()
  n255 = Release Notifier(notifier=w26, force destroy? (F)=TRUE) -> ()  [unwired: 1 in, 3 out]
